vi "Execute PC Benchmarking.vi"   [LabVIEW 2014]
uses:
  <vilib>/Utility/error.llb/DialogType.ctl
  <vilib>/Wiresmith Technology/LabVIEW CLI/CLI Class/CLI.lvclass
types:
  T1 = typedef "DialogType.ctl" = u16
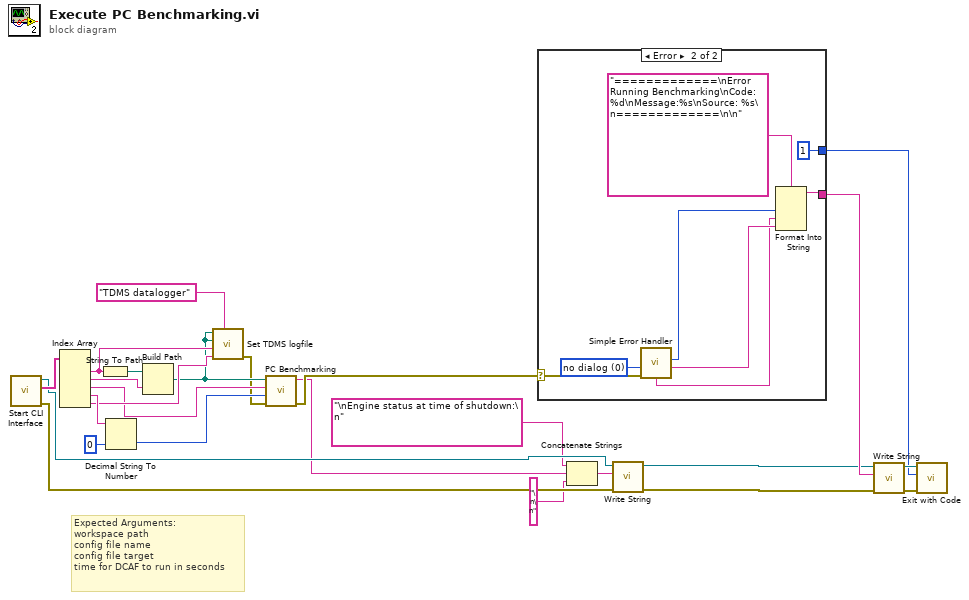
[diagram p0: block diagram]
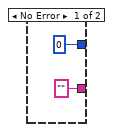
[diagram p2: hidden frame]
diagram:
  # "Expected Arguments:\nworkspace path\nconfig file name\nconfig file target\ntime for DCAF to run in seconds"
  n1 = call <vilib>:"Start CLI Interface.vi"() -> ("error out"=w8:errorcluster, "Custom Parameters"=w25:string[], "CLI out"=w6:refnum<class "CLI.lvclass">)  [unwired: 9 in]
  n2 = Index Array(array=w25) -> (element #1=w14:string, element #2=w23:string, element #3=w12:string, element #4=w18:string, element #5=w15:string)  [unwired: 5 in]
  n3 = String To Path(string=w14) -> (path=w24:path)
  n4 = Decimal String To Number(string=w18, default (0L)=u32 0 ("default (0 I32)")) -> (number=w11:u32)  [unwired: 1 in, 1 out]
  n5 = Build Path(base path=w24, name or relative path=w23) -> (appended path=w13:path)
  n6 = call "Set TDMS logfile.vi"("TDMS Module Alias"="TDMS datalogger", "log name"=w15, "Log Directory"=w14, "Config File Save Path"=w13, "Config File Path"=w13) -> ("error out"=w10:errorcluster)  [unwired: 6 in]
  n7 = call "PC Benchmarking.vi"("error in"=w10, "run time"=w11, "target alias"=w12, "configuration file path"=w13) -> ("error out"=w9:errorcluster, "engine status"=w3:string)  [unwired: 6 in]
  n8 = case shown="Error" w9 {
    selector: w9 -> [_ w32]
    tunnel: ["" w28] -> w20
    tunnel: [0 ("Exit Code (0)") 1 ("Exit Code (0)")] -> w19
    frame No Error {
    }
    frame Error {
      w33 = T1 0 items=["no dialog", "OK message", "continue or stop message", "OK message + warnings", "continue/stop + warnings"] ("type of dialog (OK msg:1)")
      n9 = call <vilib>:"Simple Error Handler.vi"("type of dialog (OK msg:1)"=w33, "error in (no error)"=w32) -> ("code out"=w31:i32, "source out"=w30:string, "message"=w29:string)  [unwired: 3 in, 2 out]
      n10 = Format Into String(format string="=============\nError Running Benchmarking\nCode: %d\nMessage:%s\nSource: %s\n=============\n\n", w31, w29, w30) -> (resulting string=w28:string)  [unwired: 2 in, 1 out]
    }
  }
  n11 = Concatenate Strings("\nEngine status at time of shutdown:\n" ("string"), w3, "\n\n" ("string")) -> (w4:string)
  n12 = call <vilib>:"Write String.vi"("error in (no error)"=w8, "Text to Write"=w4, "CLI in"=w6) -> ("error out"=w7:errorcluster, "CLI out"=w5:refnum<class "CLI.lvclass">)  [unwired: 7 in]
  n13 = call <vilib>:"Write String.vi"("error in (no error)"=w7, "Text to Write"=w20, "CLI in"=w5) -> ("error out"=w22:errorcluster, "CLI out"=w21:refnum<class "CLI.lvclass">)  [unwired: 7 in]
  n14 = call <vilib>:"Exit with Code.vi"("error in (no error)"=w22, "Exit Code (0)"=w19, "CLI in"=w21) -> ()  [unwired: 8 in, 1 out]
